vi "Launch Config Module.vi"(8 "error in (no error)":errorcluster, 11 "Volatus Core in":refnum<class "Volatus Core.lvclass">) -> (0 "error out":errorcluster, 3 "Volatus Core out":refnum<class "Volatus Core.lvclass">)   [LabVIEW 2020, in "Volatus.lvlib" / "Volatus Core.lvclass"]
uses:
  Volatus Core.lvclass
  C:/dev/lv20CE/relink/lv-volatus/Volatus/Module/Module.lvclass
  VolatusConfig/VolatusConfigElement/VolatusConfigElement.lvclass
  Config Type.ctl
  Volatus Core.lvclass/Volatus Core.ctl
  VolatusConfig/VolatusConfigElement/VolatusConfigElement.lvclass/VolatusConfigElement.ctl
  VolatusConfig/Node/Node Config.lvclass
  C:/dev/lv20CE/relink/lv-volatus/VolatusConfig/VolatusConfigElement/VolatusConfigElement.lvclass
  System Config Server/System Config Module.lvclass
  Module/Module.lvclass
  lv-cdm/CDM-Config/Config Element/Config Element.lvclass
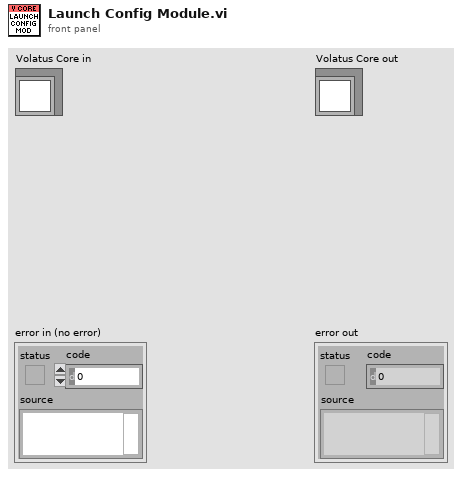
[diagram p1: front panel]
types:
  T1 = typedef "Volatus.lvlib/Volatus Core.lvclass/Config Type.ctl" = enum16{"App INI", "Memory", "Unconfigured"}
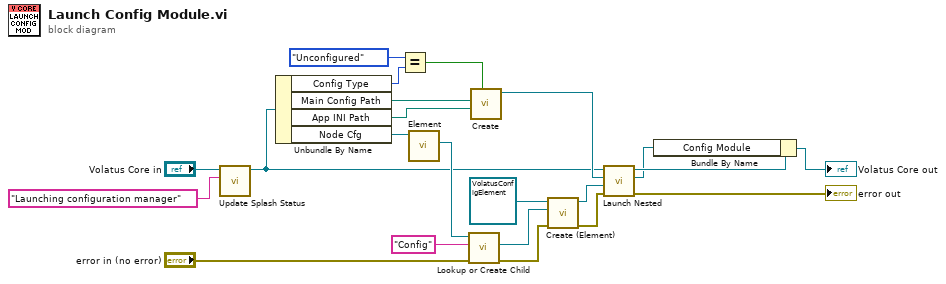
[diagram p0: block diagram]
diagram:
  n1 = call "Update Splash Status.vi"("Status"="Launching configuration manager", "Volatus Core in"="Volatus Core in") -> ("Volatus Core out"=w2:refnum<class "Volatus Core.lvclass">)  [unwired: 8 in, 1 out]
  n2 = Unbundle By Name(w2) -> ("Config Type"=w12:T1, "Main Config Path"=w17:path, "App INI Path"=w9:path, "Node Cfg"=w4:refnum<class "Node Config.lvclass">)
  n3 = Equal?(x=Config_Type."Unconfigured", y=w12) -> (x = y?=w10:bool)
  n4 = call "Element.vi"("VolatusConfigElement in"=w4) -> ("Element"=w3:refnum<class "Config Element.lvclass">)  [unwired: 9 in, 1 out]
  n5 = call "Lookup or Create Child.vi"("error in (no error)"="error in (no error)", "Name"="Config" ("Child Name"), "Config Element in"=w3) -> ("error out"=w7:errorcluster, "Child"=w6:refnum<class "Config Element.lvclass">)  [unwired: 5 in, 2 out]
  n6 = call "Create.vi"("Unconfigured"=w10, "INI Path"=w9, "Config Path"=w17) -> ("System Config Module out"=w16:refnum<class "System Config Module.lvclass">)  [unwired: 7 in, 1 out]
  n7 = call "Create (Element).vi"("error in (no error)"=w7, "Element"=w6, "VolatusConfigElement in"=refnum<class "VolatusConfigElement.lvclass"> refnum) -> ("error out"=w14:errorcluster, "VolatusConfigElement out"=w13:refnum<class "VolatusConfigElement.lvclass">)  [unwired: 7 in]
  n8 = call "Launch Nested.vi"("error in (no error)"=w14, "Config Element"=w13, "Nested Module"=w16, "Parent in"=w2) -> ("error out"=→"error out":errorcluster, "MessageQ"=w19:refnum<class "MessageQ.lvclass">, "Parent out"=w22:refnum<class "Volatus Core.lvclass">)  [unwired: 5 in]
  n9 = Bundle By Name(cluster=w22, "Config Module"=w19) -> (→"Volatus Core out":refnum<class "Volatus Core.lvclass">)
